vi "NanonisIsScanRunning.vi"(8 "error in (no error)":errorcluster, 11 "String input":string="string test") -> (0 "error out":errorcluster, 3 "String output":string)   [LabVIEW 2011]
uses:
  <userlib>/Nanonis Prog Interface/Nanonis Prog Interface.lvlib
panel:
  out "Application ref out":refnum<vi>
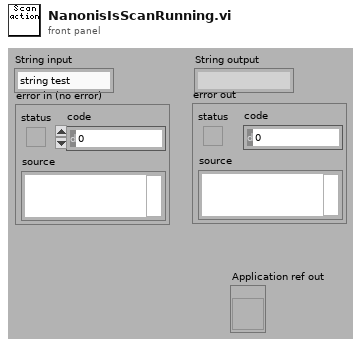
[diagram p1: front panel]
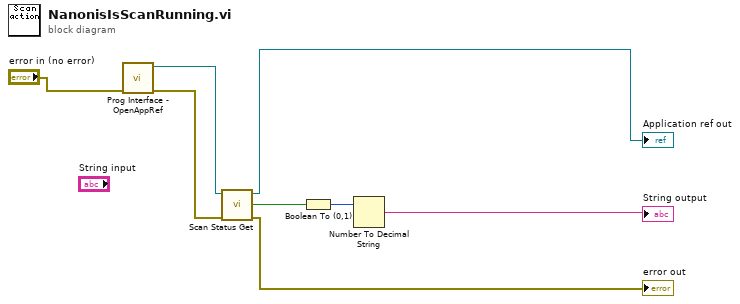
[diagram p0: block diagram]
diagram:
  n1 = call <userlib>:"Prog Interface - OpenAppRef.vi"("Error in (no error)"="error in (no error)") -> ("Error out"=w1:errorcluster, "Application reference"=w3:refnum<vi>)  [unwired: 5 in]
  n2 = call <userlib>:"Scan Status Get.vi"("error in (no error)"=w1, "Application ref in"=w3) -> ("error out"=→"error out":errorcluster, "Scanning?"=w7:bool, "Application ref out"=→"Application ref out":refnum<vi>)  [unwired: 6 in]
  n3 = Boolean To (0,1)(Boolean=w7) -> (0, 1=w5:i16)
  n4 = Number To Decimal String(number=w5) -> (decimal integer string=→"String output":string)  [unwired: 1 in]
